vi "Wake Up HL.vi"(4 "frequency":dbl, 5 "signal type":T1(ring), 6 "offset":dbl, 7 "amplitude":dbl, 8 "error in":errorcluster, 9 "phase":dbl, 10 "Timeout":i32, 11 "Module ID":i32=-1) -> (0 "error out":errorcluster)   [LabVIEW 2026, in "Function Generator.lvlib"]
doc: "_____\nCreated using DQMH Framework: Event Scripter 7.1.2.1547."
uses:
  Function Generator.lvlib
  Wake Up HL Argument--cluster.ctl
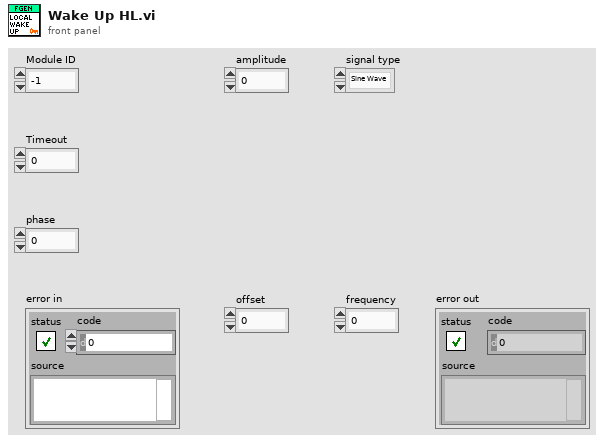
[diagram p1: front panel]
types:
  T1 = enum16{"Sine Wave", "Triangle Wave", "Square Wave", "Sawtooth Wave"}
  T2 = typedef "Function Generator.lvlib/Wake Up HL Argument--cluster.ctl" = cluster{"Module ID":i32, "Timeout":i32, "signal type":enum16{"Sine Wave", "Triangle Wave", "Square Wave", "Sawtooth Wave"}, "amplitude":dbl, "phase":dbl, "frequency":dbl, "offset 2":dbl}
  T3 = typedef "Function Generator.lvlib/Request Events--cluster.ctl" = cluster{"Stop Module":refnum<user-event>, "Show Panel":refnum<user-event>, "Hide Panel":refnum<user-event>, "Show Diagram":refnum<user-event>, "Get Module Execution Status":refnum<user-event>, "Set Signal Type":refnum<user-event>, "Set Signal Parameters":refnum<user-event>, "Start":refnum<user-event>, "Local Instance":T4}
  T4 = typedef "Function Generator.lvlib/Local Instance Request Events--cluster.ctl" = cluster{"Wake Up HL":refnum<user-event>}
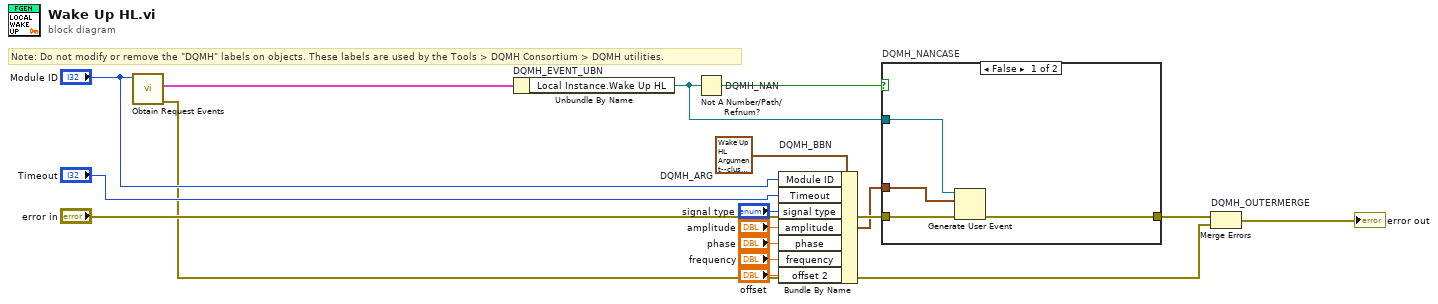
[diagram p0: block diagram]
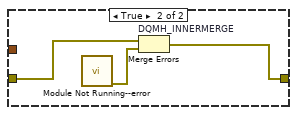
[diagram p2: hidden frame]
diagram:
  w10 = T2 {"Module ID"=-1, "Timeout"=0, "signal type"=enum."Sine Wave", "amplitude"=1.0, "phase"=0.0, "frequency"=10.0, "offset 2"=0.0}  # DQMH_ARG
  # "Note: Do not modify or remove the \"DQMH\" labels on objects. These labels are used by the Tools > DQMH Consortium > DQMH utilities."
  n1 = call "Obtain Request Events.vi"("Module ID"="Module ID") -> ("error out"=w7:errorcluster, "Function Generator Request Events"=w6:T3)  [unwired: 9 in]
  n2 = Unbundle By Name "DQMH_EVENT_UBN"(w6) -> ("Local Instance.Wake Up HL"=w12:refnum<user-event>)
  n3 = Not A Number/Path/Refnum? "DQMH_NAN"(number/path/refnum=w12) -> (NaN/Path/Refnum?=w13:bool)
  n4 = Bundle By Name "DQMH_BBN"(cluster=w10, "Module ID"="Module ID", "Timeout"="Timeout", "signal type"="signal type", "amplitude"="amplitude", "phase"="phase", "frequency"="frequency", "offset 2"="offset") -> (w14:T2)
  n5 = case "DQMH_NANCASE" shown="False" w13 {
    tunnel: "error in" -> [w20 w23]
    tunnel: [w19 w22] -> w11
    tunnel: w12 -> [w18 _]
    tunnel: w14 -> [w17 _]
    frame False {
      n6 = Generate User Event(user event=w18, event data cluster=w17, error in=w20) -> (error out=w19:errorcluster)  [unwired: 1 in, 1 out]
    }
    frame True {
      n7 = call "Module Not Running--error.vi"() -> ("error out"=w21:errorcluster)  [unwired: 11 in]
      n8 = Merge Errors "DQMH_INNERMERGE"(w23, w21) -> (w22:errorcluster)
    }
  }
  n9 = Merge Errors "DQMH_OUTERMERGE"(w11, w7) -> (→"error out":errorcluster)
